vi "RPC Method ThermalChamberController StartModule.vi"(8 "error in (no error)":errorcluster, 11 "gRPC service in":refnum<class "ThermalChamberController.lvclass">) -> (0 "error out":errorcluster, 3 "gRPC service out":refnum<class "ThermalChamberController.lvclass">)   [LabVIEW 2020, in "thermal-chamber-controller_server.lvlib" / "ThermalChamberController.lvclass"]
uses:
  ThermalChamberController.lvclass
  ThermalChamberController.lvclass/ThermalChamberController.ctl
  RPC Messages/lv_python_grpc_webui_demo_v1_Empty.ctl
  Program Files (x86)/National Instruments/LabVIEW 2020/examples/DQMH Consortium/DQMH Fundamentals - Thermal Chamber/Libraries/Thermal Chamber Controller_DQMH/Thermal Chamber Controller_DQMH.lvlib
  thermal-chamber-controller_server.lvlib
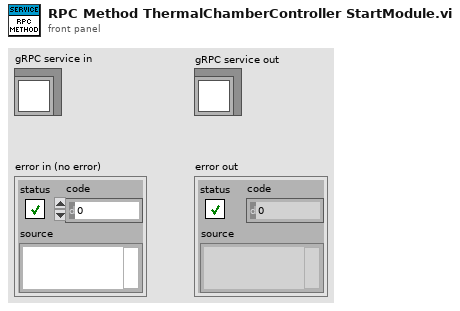
[diagram p1: front panel]
types:
  T1 = typedef "thermal-chamber-controller_server.lvlib/lv_python_grpc_webui_demo_v1_Empty.ctl" = cluster{"void":string}
  T2 = typedef "thermal-chamber-controller_server.lvlib/ThermalChamberController.lvclass/Server Internal UEs.ctl" = cluster{"ThermalChamberController StartModule Internal UE":refnum<user-event>, "ThermalChamberController ShowModulePanel Internal UE":refnum<user-event>, "ThermalChamberController HideModulePanel Internal UE":refnum<user-event>, "ThermalChamberController StopModule Internal UE":refnum<user-event>, "ThermalChamberController UpdateSetPoint Internal UE":refnum<user-event>, "ThermalChamberController UpdateRampRate Internal UE":refnum<user-event>, "ThermalChamberController UpdateHeaterState Internal UE":refnum<user-event>, "ThermalChamberController SubscribeChamberStatusUpdated Internal UE":refnum<user-event>, "ThermalChamberController SubscribeSetPointUpdated Internal UE":refnum<user-event>, "ThermalChamberController SubscribeRampRateUpdated Internal UE":refnum<user-event>, "ThermalChamberController SubscribeHeaterStateUpdated Internal UE":refnum<user-event>}
  T3 = typedef "thermal-chamber-controller_server.lvlib/ThermalChamberController.lvclass/Server gRPC UEs.ctl" = cluster{"ThermalChamberController StartModule gRPC UE":refnum<user-event>, "ThermalChamberController ShowModulePanel gRPC UE":refnum<user-event>, "ThermalChamberController HideModulePanel gRPC UE":refnum<user-event>, "ThermalChamberController StopModule gRPC UE":refnum<user-event>, "ThermalChamberController UpdateSetPoint gRPC UE":refnum<user-event>, "ThermalChamberController UpdateRampRate gRPC UE":refnum<user-event>, "ThermalChamberController UpdateHeaterState gRPC UE":refnum<user-event>, "ThermalChamberController SubscribeChamberStatusUpdated gRPC UE":refnum<user-event>, "ThermalChamberController SubscribeSetPointUpdated gRPC UE":refnum<user-event>, "ThermalChamberController SubscribeRampRateUpdated gRPC UE":refnum<user-event>, "ThermalChamberController SubscribeHeaterStateUpdated gRPC UE":refnum<user-event>}
  T4 = typedef "Thermal Chamber Controller_DQMH.lvlib/Broadcast Events--cluster.ctl" = cluster{"Module Did Init":refnum<user-event>, "Status Updated":refnum<user-event>, "Error Reported":refnum<user-event>, "Module Did Stop":refnum<user-event>, "Update Module Execution Status":refnum<user-event>, "Chamber Status Updated":refnum<user-event>, "Set Point Updated":refnum<user-event>, "Ramp Rate Updated":refnum<user-event>, "Heater State Updated":refnum<user-event>}
  T5 = typedef "grpc-lvsupport-release.lvlib/grpcId.ctl" = u64
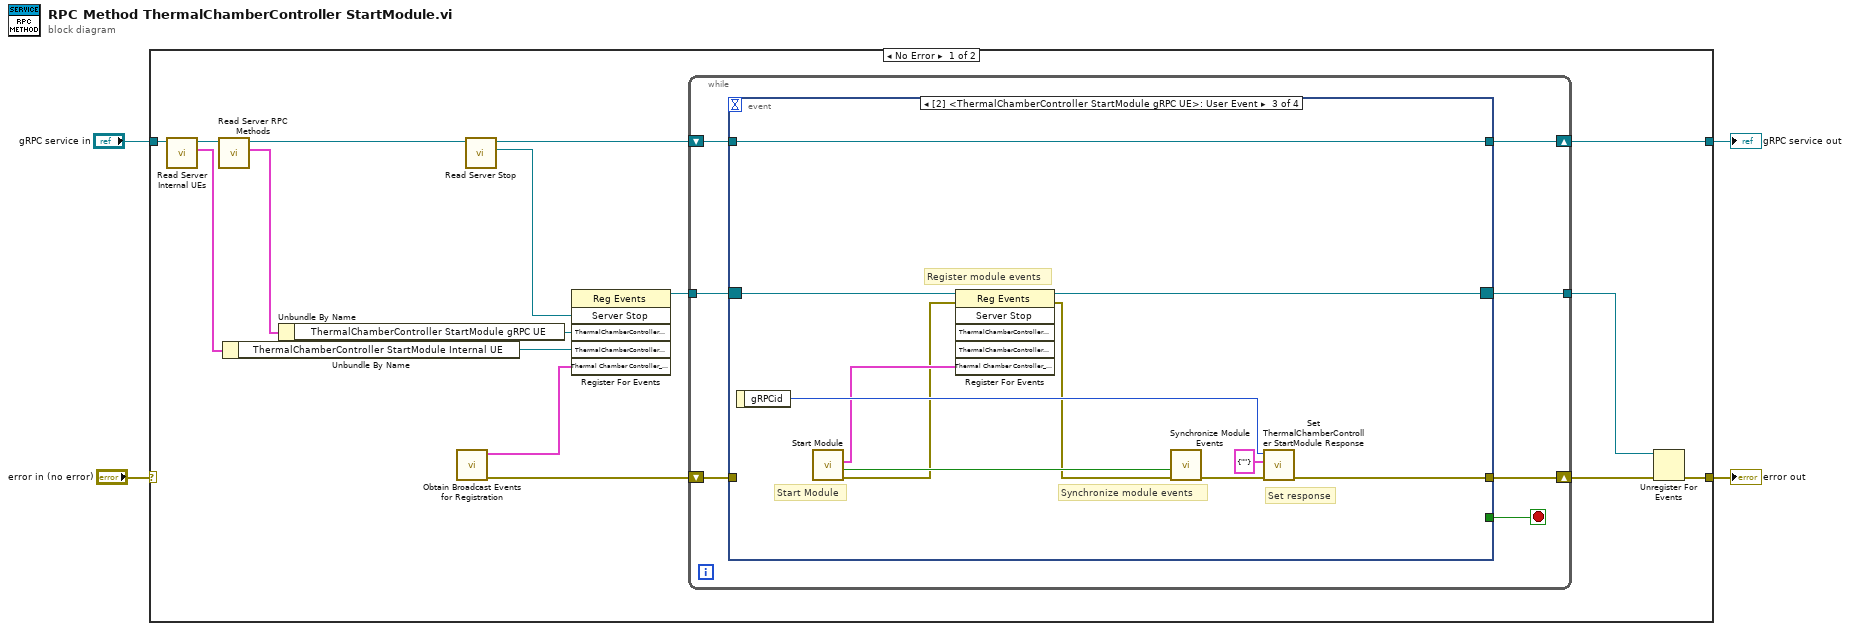
[diagram p0: block diagram]
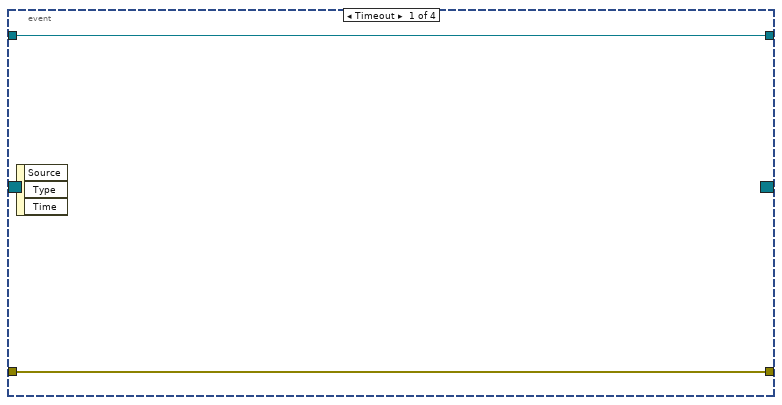
[diagram p2: hidden frame]
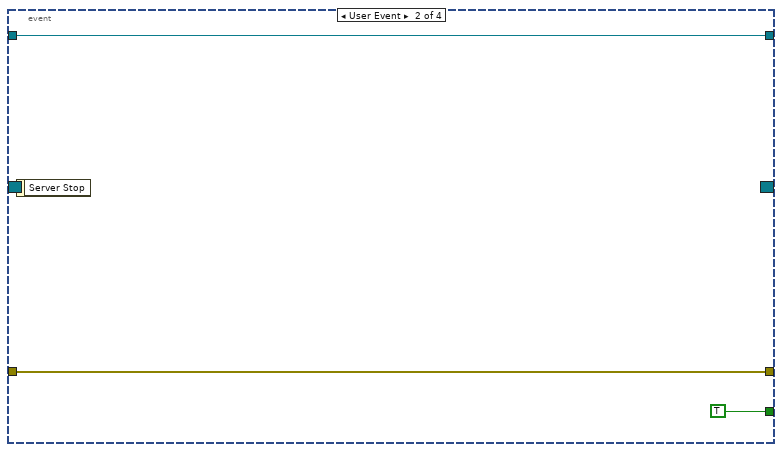
[diagram p3: hidden frame]
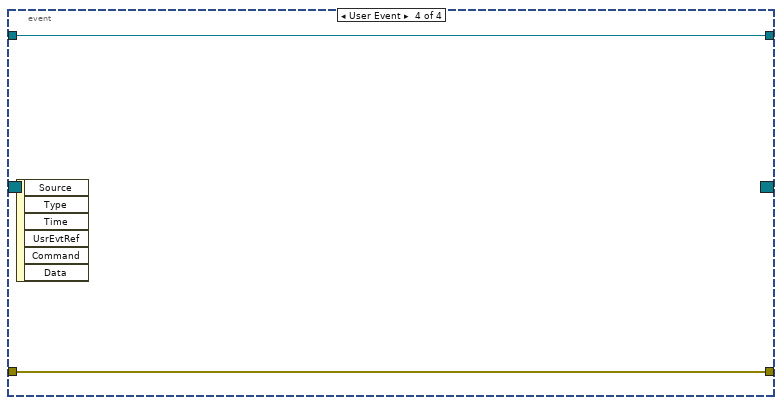
[diagram p4: hidden frame]
diagram:
  n1 = case shown="No Error" "error in (no error)" {
    selector: "error in (no error)" -> [_ w47]
    tunnel: [w15 w47] -> w3
    tunnel: "gRPC service in" -> [w18 w46]
    tunnel: [w7 w46] -> w1
    frame No Error {
      n2 = call "Read Server Internal UEs.vi"("gRPC service in"=w18) -> ("Server Internal UEs"=w11:T2, "gRPC service out"=w17:refnum<class "ThermalChamberController.lvclass">)  [unwired: 8 in, 1 out]
      n3 = call "Read Server RPC Methods.vi"("gRPC service in"=w17) -> ("Server RPC Methods"=w13:T3, "gRPC service out"=w8:refnum<class "ThermalChamberController.lvclass">)  [unwired: 8 in, 1 out]
      n4 = Unbundle By Name ("Unbundle Internal UE")(w11) -> ("ThermalChamberController StartModule Internal UE"=w10:refnum<user-event>)
      n5 = Unbundle By Name ("Unbundle gRPC UE")(w13) -> ("ThermalChamberController StartModule gRPC UE"=w12:refnum<user-event>)
      n6 = call "Obtain Broadcast Events for Registration.vi"() -> ("error out"=w6:errorcluster, "Thermal Chamber Controller_DQMH Broadcast Events"=w5:T4)  [unwired: 9 in, 1 out]
      n7 = call-dynamic "Read Server Stop.vi"("gRPC service in"=w8) -> ("Server Stop"=w20:refnum<user-event>, "gRPC service out"=w9:refnum<class "ThermalChamberController.lvclass">)  [unwired: 8 in, 1 out]
      n8 = register-events(w20, w12, w10, w5) -> (reference out=w19:refnum<event-registration>)  [unwired: 2 in, 1 out]
      n9 = while {
        tunnel: w19 -> [w27]
        tunnel: [w23] -> w14
        shift-right: [w24] -> w16
        shift-left: w6 -> [w25]
        shift-right: [w21] -> w7
        shift-left: w9 -> [w22]
        stop <- w26 stop-if-true
        n10 = event "RPC Method Event Structure" shown="[2] <ThermalChamberController StartModule gRPC UE>: User Event" {
          selector: w27 -> [_ _ w38 _]
          dyn-events: [_ _ w34 _] -> w23
          timeout: _ -> [_ _ _ _]
          tunnel: [_ TRUE _ _] -> w26
          tunnel: w25 -> [w29 w31 _ w45]
          tunnel: [w29 w31 w40 w45] -> w24
          tunnel: w22 -> [w28 w30 w43 w44]
          tunnel: [w28 w30 w43 w44] -> w21
          event Timeout {
            n11 = event-data() -> ()  [unwired: 1 in, 3 out]
          }
          event User Event {
            n12 = event-data() -> ()  [unwired: 1 in, 1 out]
          }
          event User Event {
            # "Set response"
            # "Synchronize module events"
            # "Register module events"
            # "Start Module"
            n13 = event-data() -> ("gRPCid"=w39:T5)  [unwired: 1 in]
            n14 = call "Start Module.vi"() -> ("error out"=w36:errorcluster, "Wait for Event Sync?"=w42:bool, "Thermal Chamber Controller_DQMH Broadcast Events"=w37:T4)  [unwired: 7 in, 2 out]
            n15 = register-events(reference=w38, error in=w36, w37) -> (reference out=w34:refnum<event-registration>, error out=w35:errorcluster)  [unwired: 3 in]
            n16 = call "Synchronize Module Events.vi"("error in"=w35, "Wait for Event Sync?"=w42) -> ("error out"=w41:errorcluster)  [unwired: 9 in]
            n17 = call "Set ThermalChamberController StartModule Response.vi"("error in (no error)"=w41, "Message Data"=T1 {"void"=""}, "gRPCid in"=w39) -> ("error out"=w40:errorcluster)  [unwired: 8 in]
          }
          event User Event {
            n18 = event-data() -> ()  [unwired: 1 in, 6 out]
          }
        }
      }
      n19 = Unregister For Events(event registration refnum=w14, error in=w16) -> (error out=w15:errorcluster)
    }
    frame Error {
    }
  }
  "error out" <- w3
  "gRPC service out" <- w1
